vi "Get Vendor Name.vi"(8 "error in (no error)":errorcluster, 9 "LARGO":u32, 10 "VARIBLE":string, 11 "HANDLE":u32) -> (0 "error out":errorcluster, 2 "NOMBRE":string, 3 "OUT":u32)   [LabVIEW 2011, in "HID_ARZ.lvlib"]
doc: "GET_VENDOR_NAME GetVendorName;"
uses:
  HID_ARZ.lvlib
  <userlib>/HID_ARZ/mcHID.dll
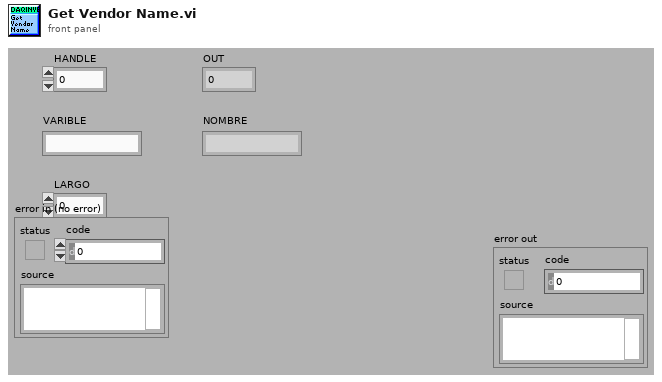
[diagram p1: front panel]
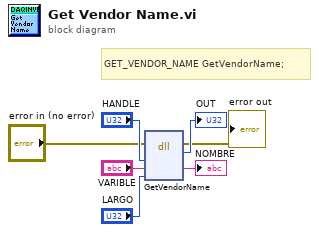
[diagram p0: block diagram]
diagram:
  # "GET_VENDOR_NAME GetVendorName;"
  n1 = dll-call lib="C:/Program Files (x86)/National Instruments/LabVIEW 2017/user.lib/HID_ARZ/mcHID.*" fn="GetVendorName"(error in="error in (no error)", "para0"="HANDLE", "para1"="VARIBLE", "para2"="LARGO") -> (error out=→"error out":errorcluster, "return type"=→"OUT":u32, "para1"=→"NOMBRE":string)  [unwired: 4 in, 1 out]
